vi "OwnOop20261013_CreateAccessorsV2.vi"() -> ()   [LabVIEW 2024]
uses:
  <resource>/Framework/Providers/LVClassLibrary/NewAccessors/MemberVICreation.lvlib
  <resource>/Framework/Providers/LVClassLibrary/NewAccessors/CLSUIP_Access.ctl
panel:
  out "error out":errorcluster caption="错误输出"
  in  "Write Path Without Diagram":bool
  in  "Write Path Save a Copy":bool
  in  "Write Path":path
  in  "Read Path Without Diagram":bool
  in  "Read Path Save a Copy":bool
  in  "Read Path":path
  in  "Virtual Folder Name":string
  in  "PDC Item Refnum":refnum<vi>
  in  "Make available through Property Nodes":bool
  in  "Include error terminals":bool
  in  "Access UI":T1
  in  "VI Type":enum32{"Dynamic", "Static"}(ring)=enum."Static"
  in  "Class Path":path
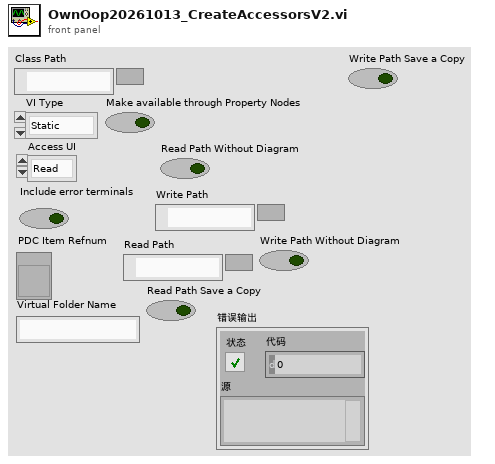
[diagram p1: front panel]
types:
  T1 = typedef "MemberVICreation.lvlib/CLSUIP_Access.ctl" = enum16{"Read", "Write", "R/W"}
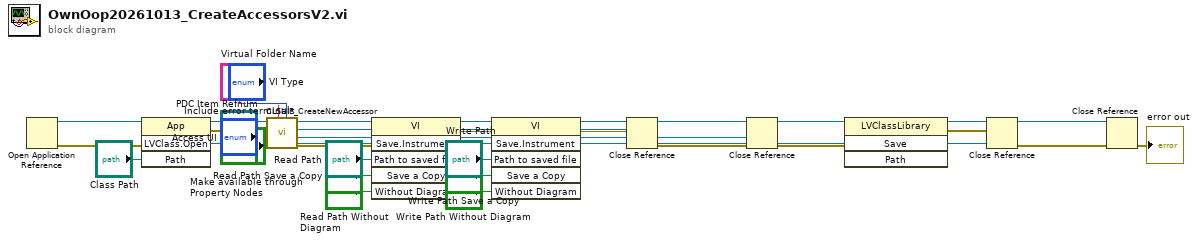
[diagram p0: block diagram]
diagram:
  n1 = Open Application Reference() -> (0:w25:errorcluster, 3:w27:refnum<vi>)  [unwired: 4 in]
  n2 = invoke class="App" method="LVClass.Open"(reference=w27, error in=w25, "Path"="Class Path") -> (error out=w23:errorcluster, "LVClass.Open"=w24:refnum<vi>)  [unwired: 1 in, 2 out]
  n3 = call <resource>:"CLSUIP_CreateNewAccessor.vi"("Make available through Property Nodes"="Make available through Property Nodes", "VI Type"="VI Type", "Include error terminals"="Include error terminals", "Virtual Folder Name"="Virtual Folder Name", "error in (no error)"=w23, "Access UI"="Access UI", "PDC Item Refnum"="PDC Item Refnum", "LVClassLibrary Ref"=w24) -> ("error out"=w12:errorcluster, "Write VI"=w11:refnum<vi>, "Read VI"=w16:refnum<vi>)  [unwired: 1 in]
  n4 = invoke class="VI" method="Save.Instrument"(reference=w16, error in=w12, "Path to saved file"="Read Path", "Save a Copy"="Read Path Save a Copy", "Without Diagram"="Read Path Without Diagram") -> (error out=w7:errorcluster)  [unwired: 1 in, 5 out]
  n5 = invoke class="VI" method="Save.Instrument"(reference=w11, error in=w7, "Path to saved file"="Write Path", "Save a Copy"="Write Path Save a Copy", "Without Diagram"="Write Path Without Diagram") -> (error out=w6:errorcluster)  [unwired: 1 in, 5 out]
  n6 = Close Reference(reference=w16, error in (no error)=w6) -> (error out=w5:errorcluster)
  n7 = Close Reference(reference=w11, error in (no error)=w5) -> (error out=w4:errorcluster)
  n8 = invoke class="LVClassLibrary" method="Save"(reference=w24, error in=w4) -> (error out=w3:errorcluster)  [unwired: 2 in, 3 out]
  n9 = Close Reference(reference=w24, error in (no error)=w3) -> (error out=w2:errorcluster)
  n10 = Close Reference(reference=w27, error in (no error)=w2) -> (error out=→"error out":errorcluster)
